vi "ZM-CP-publish.vi"(8 "error in (no error)":errorcluster, 10 "package":refnum<class "ZM-PC-package.lvclass">, 11 "ZM-CP-communication_protocol in":refnum<class "ZM-CP-communication_protocol.lvclass">) -> (0 "error out":errorcluster, 3 "ZM-CP-communication_protocol out":refnum<class "ZM-CP-communication_protocol.lvclass">)   [LabVIEW 2020, in "ZM-CP-communication_protocol.lvlib" / "ZM-CP-communication_protocol.lvclass"]
doc: "Placeholder: returns error 5000 (#customerror 5000). A child class must override it and publish the package it is given. The package input (a ZM-PC-package) is not used here; the error is built by Bundle By Name onto an error-cluster constant (status TRUE, code 5000, source ZM-CP-publish.vi: must be overridden by a child class) and merged after error in, so an incoming error wins."
uses:
  ZM-CP-communication_protocol.lvclass
  common/ZM-PC-packages/ZM-PC-package/ZM-PC-package.lvclass
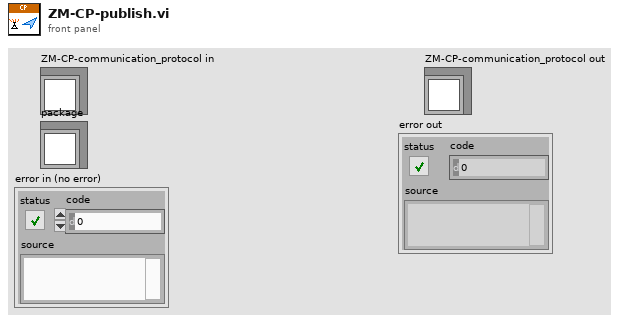
[diagram p1: front panel]
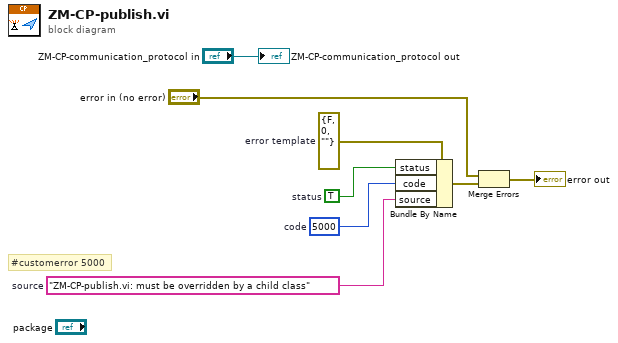
[diagram p0: block diagram]
diagram:
  w6 = "ZM-CP-publish.vi: must be overridden by a child class"  # source
  w7 = 5000  # code
  w8 = TRUE  # status
  w5 = errorcluster {"status"=FALSE, "code"=0, "source"=""}  # error template
  # "#customerror 5000"
  n1 = Bundle By Name(cluster=w5, "status"=w8, "code"=w7, "source"=w6) -> (w3:errorcluster)
  n2 = Merge Errors("error in (no error)", w3) -> (→"error out":errorcluster)
  "ZM-CP-communication_protocol out" <- "ZM-CP-communication_protocol in"
